vi "Update Measurement Selection.vi"(8 "error in (no error)":errorcluster, 10 "mouseDown coords":T1, 11 "multicolumnListbox in":refnum<vi>) -> (0 "error out":errorcluster, 3 "multicolumnListbox out":refnum<vi>)   [LabVIEW 2021, in "MeasurementClient Editor.lvlib"]
uses:
  MeasurementClient Editor.lvlib
  <vilib>/Utility/miscctls.llb/LVPoint32TypeDef.ctl
  <vilib>/Utility/miscctls.llb/LVPositionTypeDef.ctl
  <vilib>/Utility/miscctls.llb/LVRowAndColumnTypeDef.ctl
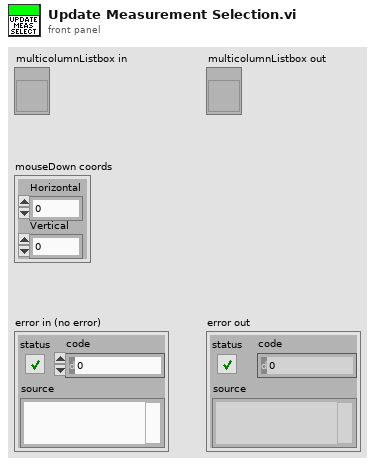
[diagram p1: front panel]
types:
  T1 = typedef "LVPoint32TypeDef.ctl" = cluster{"Horizontal":i32, "Vertical":i32}
  T2 = typedef "LVPositionTypeDef.ctl" = cluster{"Left":i32, "Top":i32}
  T3 = typedef "LVRowAndColumnTypeDef.ctl" = cluster{"Row":i32, "Column":i32}
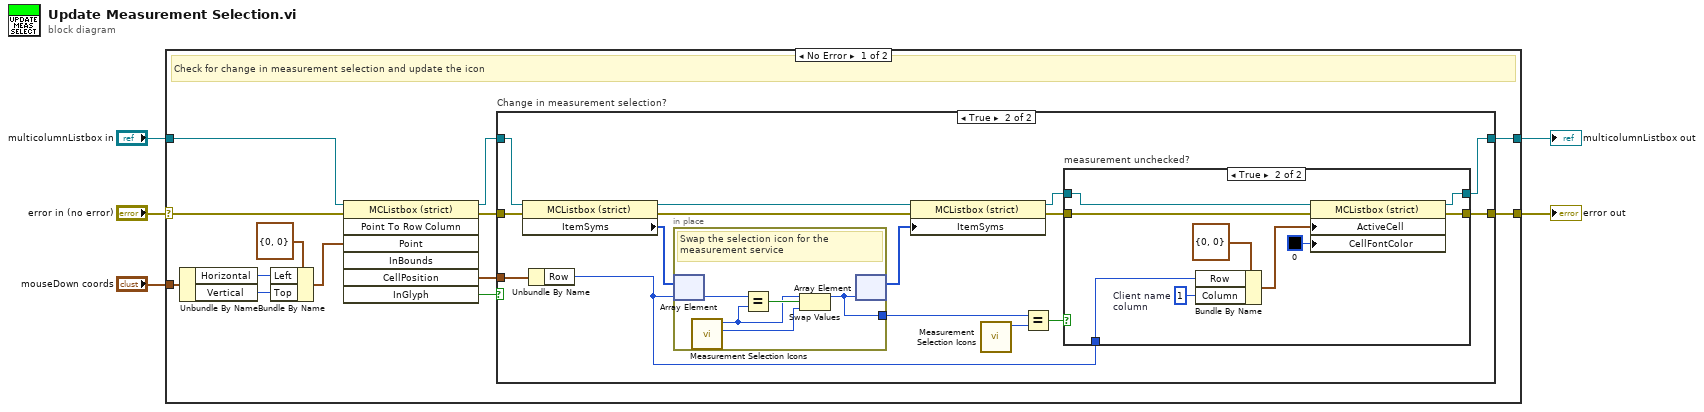
[diagram p0: block diagram]
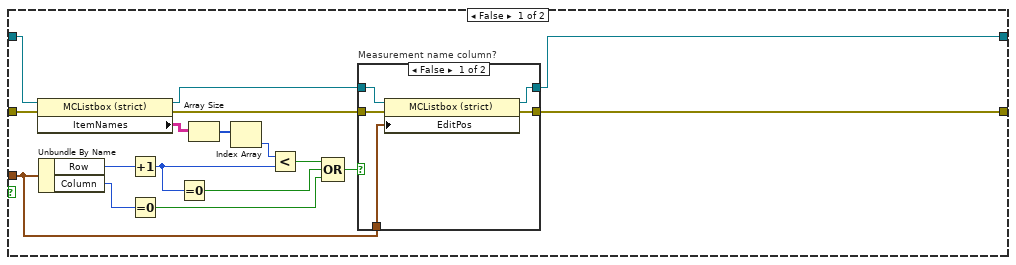
[diagram p2: hidden frame]
diagram:
  n1 = case shown="No Error" "error in (no error)" {
    selector: "error in (no error)" -> [w13 w74]
    tunnel: [w18 w74] -> w5
    tunnel: [w7 w75] -> w4
    tunnel: "multicolumnListbox in" -> [w14 w75]
    tunnel: "mouseDown coords" -> [w12 _]
    frame No Error {
      # "Check for change in measurement selection and update the icon"
      n2 = Unbundle By Name(w12) -> ("Horizontal"=w9:i32, "Vertical"=w8:i32)
      n3 = Bundle By Name(cluster=T2 {"Left"=0, "Top"=0} ("Point"), "Left"=w9, "Top"=w8) -> (w10:T2)
      n4 = invoke class="MCListbox (strict)" method="Point To Row Column"(reference=w14, error in=w13, "Point"=w10) -> (reference out=w17:refnum<vi>, error out=w15:errorcluster, "CellPosition"=w16:T3, "InGlyph"=w6:bool)  [unwired: 4 in, 3 out]
      n5 = case "Change in measurement selection?" shown="True" w6 {
        tunnel: w15 -> [w28 w57]
        tunnel: w16 -> [w24 w55]
        tunnel: w17 -> [w27 w56]
        tunnel: [w26 w43] -> w7
        tunnel: [w25 w47] -> w18
        frame False {
          n6 = property class="MCListbox (strict)"(reference=w27, error in=w28) -> (reference out=w29:refnum<vi>, error out=w34:errorcluster, "ItemNames"=w33:string[][])
          n7 = Unbundle By Name(w24) -> ("Row"=w30:i32, "Column"=w35:i32)
          n8 = Increment(x=w30) -> (x+1=w23:i32)
          n9 = Equal To 0?(x=w35) -> (x = 0?=w21:bool)
          n10 = Equal To 0?(x=w23) -> (x = 0?=w22:bool)
          n11 = Array Size(array=w33) -> (size(s)=w32:i32[])
          n12 = Index Array(array=w32) -> (element=w31:i32)  [unwired: 1 in]
          n13 = Less?(x=w31, y=w23) -> (x < y?=w20:bool)
          n14 = Compound Arithmetic op=OR(w20, w22, w21) -> (w19:bool)
          n15 = case "Measurement name column?" shown="False" w19 {
            tunnel: w34 -> [w40 w42]
            tunnel: [w39 w42] -> w25
            tunnel: [w38 w41] -> w26
            tunnel: w29 -> [w37 w41]
            tunnel: w24 -> [w36 _]
            frame False {
              n16 = property class="MCListbox (strict)"(reference=w37, error in=w40, "EditPos"=w36) -> (reference out=w38:refnum<vi>, error out=w39:errorcluster)
            }
            frame True {
            }
          }
        }
        frame True {
          n17 = property class="MCListbox (strict)"(reference=w56, error in=w57) -> (reference out=w54:refnum<vi>, error out=w53:errorcluster, "ItemSyms"=w52:i32[])
          n18 = Unbundle By Name(w55) -> ("Row"=w44:i32)
          n19 = in-place {
            in-place-border: [w69] -> w50
            # "Swap the selection icon for the measurement service"
            n20 = in-place-array #1(w52, w44) -> (w73:i32)
            n21 = call "Measurement Selection Icons.vi"() -> ("Checked"=w70:i32, "Unchecked"=w71:i32)  [unwired: 10 in]
            n22 = Equal?(x=w73, y=w71) -> (x = y?=w72:bool)
            n23 = Swap Values(12:w71, 13:w72, 14:w70) -> (1:w69:i32)  [unwired: 1 out]
            n24 = in-place-array #1(w69) -> (w51:i32[])  [unwired: 1 out]
          }
          n25 = property class="MCListbox (strict)"(reference=w54, error in=w53, "ItemSyms"=w51) -> (reference out=w45:refnum<vi>, error out=w48:errorcluster)
          n26 = call "Measurement Selection Icons.vi"() -> ("Unchecked"=w49:i32)  [unwired: 10 in, 1 out]
          n27 = Equal?(x=w50, y=w49) -> (x = y?=w46:bool)
          n28 = case "measurement unchecked?" shown="True" w46 {
            tunnel: w48 -> [w59 w68]
            tunnel: [w59 w67] -> w47
            tunnel: w45 -> [w58 w66]
            tunnel: w44 -> [_ w63]
            tunnel: [w58 w60] -> w43
            frame False {
            }
            frame True {
              w64 = 1  # Client name column
              n29 = Bundle By Name(cluster=T3 {"Row"=0, "Column"=0} ("Active Cell:Active Cell"), "Row"=w63, "Column"=w64) -> (w62:T3)
              n30 = property class="MCListbox (strict)"(reference=w66, error in=w68, "ActiveCell"=w62, "CellFontColor"=u32 0 ("Active Cell:Cell Font:Color")) -> (reference out=w60:refnum<vi>, error out=w67:errorcluster)
            }
          }
        }
      }
    }
    frame Error {
      # "Pass"
    }
  }
  "error out" <- w5
  "multicolumnListbox out" <- w4
